vi "Remove Bitfile.vi"(8 "error in (no error)":errorcluster, 10 "RIO Device Address":string, 11 "EST Custom Device in":refnum<k24>) -> (0 "error out":errorcluster, 3 "EST Custom Device out":refnum<k24>)   [LabVIEW 2020, in "Engine Simulation Toolkit Scripting API.lvlib"]
uses:
  Engine Simulation Toolkit Scripting API.lvlib
  NationalInstruments.VeriStand.SystemDefinitionAPI
  Shared/Properties.vi
  <vilib>/NI VeriStand/Custom Device API/Get Item Property (String Array).vi
  System Explorer/Engine Simulation Toolkit System Explorer.lvlib
  <vilib>/NI VeriStand/Custom Device API/Custom Device API.lvlib
  Shared/Engine Simulation Toolkit Shared.lvlib
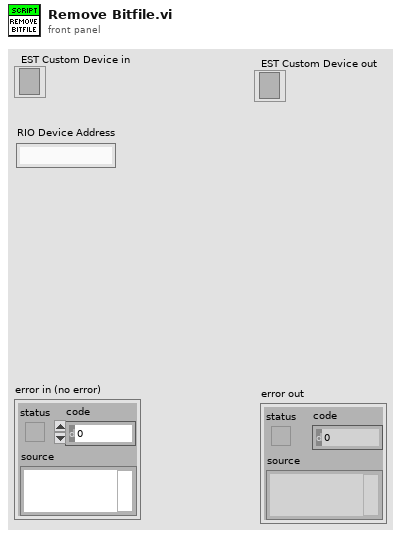
[diagram p1: front panel]
types:
  T1 = typedef "Custom Device API.lvlib/Custom Device Item Ref.ctl" = u64
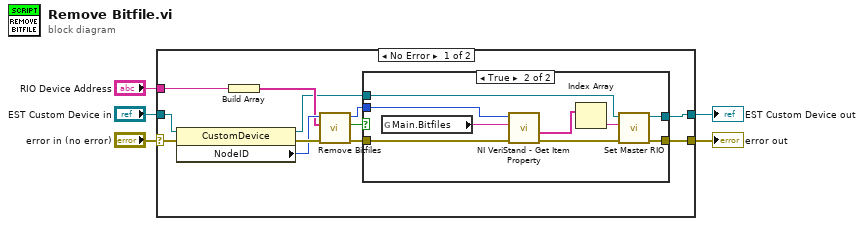
[diagram p0: block diagram]
diagram:
  n1 = case shown="No Error" "error in (no error)" {
    selector: "error in (no error)" -> [w16 w30]
    tunnel: [w14 w30] -> w5
    tunnel: "EST Custom Device in" -> [w17 w29]
    tunnel: [w15 w29] -> w2
    tunnel: "RIO Device Address" -> [w10 _]
    frame No Error {
      n2 = property class="CustomDevice"(reference=w17, error in=w16) -> (reference out=w8:refnum<k24>, error out=w13:errorcluster, "NodeID"=w12:u64)
      n3 = Build Array(w10) -> (w11:string[])
      n4 = call "Remove Bitfiles.vi"("error in (no error)"=w13, "RIO Addresses"=w11, "Item Ref in"=w12) -> ("error out"=w9:errorcluster, "Need to select a new master?"=w7:bool, "Item Ref out"=w6:T1)  [unwired: 5 in, 1 out]
      n5 = case shown="True" w7 {
        tunnel: [w18 w28] -> w15
        tunnel: w9 -> [w19 w23]
        tunnel: [w19 w27] -> w14
        tunnel: w8 -> [w18 w26]
        tunnel: w6 -> [_ w24]
        frame False {
        }
        frame True {
          n6 = global read "Properties.vi" "Main.Bitfiles"() -> (w25:string)
          n7 = call-poly <vilib>:"NI VeriStand - Get Item Property.vi"("error in (no error)"=w23, "Property Name"=w25, "Item Ref in"=w24) -> ("error out"=w22:errorcluster, "Value"=w21:string[])  [unwired: 5 in, 2 out]
          n8 = Index Array(array=w21) -> (element=w20:string)  [unwired: 1 in]
          n9 = call "Set Master RIO.vi"("error in (no error)"=w22, "RIO Device Address"=w20, "EST Custom Device in"=w26) -> ("error out"=w27:errorcluster, "EST Custom Device out"=w28:refnum<k24>)  [unwired: 7 in]
        }
      }
    }
    frame Error {
    }
  }
  "EST Custom Device out" <- w2
  "error out" <- w5
